vi "Kinect MAIN.vi"() -> ()   [LabVIEW 2014]
uses:
  Resources/Others/Control cluster.ctl
  <vilib>/University of Leeds/Kinesthesia Toolkit for Microsoft Kinect/_Polymorphic Configure/Event-Skeleton and Video.vi
  Kinect Global.vi
  <vilib>/University of Leeds/Kinesthesia Toolkit for Microsoft Kinect/_Polymorphic Read/Read-Skeleton and Video.vi
  <vilib>/University of Leeds/Kinesthesia Toolkit for Microsoft Kinect/_Polymorphic Close/Close-Skeleton and Video.vi
panel:
  out "Toggle Land/Take off":bool
  out "Hover":bool
  out "Control Cluster out":T1 {"Yaw Speed" scale=-1.0..1.0; "Vertical Speed" scale=-1.0..1.0; "Pitch" scale=-1.0..1.0; "Roll" scale=-1.0..1.0}
  out "pitch offset":dbl=0.15 format="%#_13g"
  out "Weak detect":bool=TRUE
  out "Colour data":picture
  out "error out":errorcluster
  out "Loop time":u32=25
  out "3D Picture":refnum<vi>(3d-picture)
  in  "stop":bool
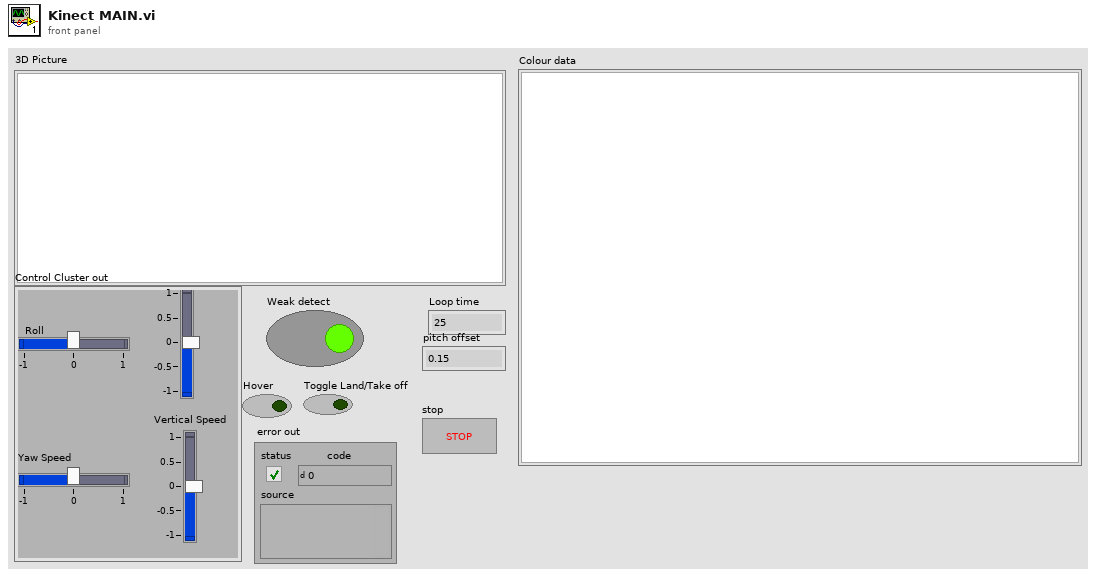
[diagram p1: front panel]
types:
  T1 = typedef "Control cluster.ctl" = cluster{"Roll":sgl, "Pitch":sgl, "Vertical Speed":sgl, "Yaw Speed":sgl}
  T2 = cluster{cluster{"reference out":refnum<k24>, "KinectSensors":refnum<k24>}, "get_Item":refnum<k24>}
  T3 = cluster{"Scene":refnum<vi>, "Joints":refnum<vi>[], "Bones":refnum<vi>[]}
  T4 = cluster{"reference out":refnum<k24>, "KinectSensors":refnum<k24>, "SkeletonStream":refnum<k24>, "ColorStream":refnum<k24>, refnum<k24>[], "get_Item":refnum<k24>}
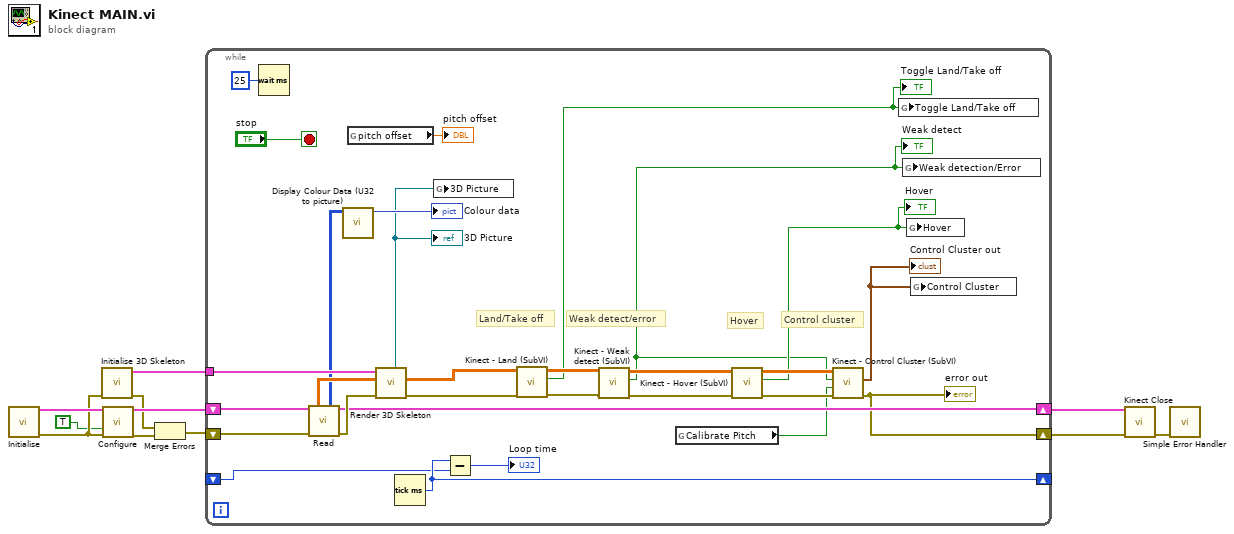
[diagram p0: block diagram]
diagram:
  n1 = call <vilib>:"Initialise.vi"() -> ("Kinect References out"=w11:T2, "error out"=w7:errorcluster)  [unwired: 14 in]
  n2 = call <vilib>:"Initialise 3D Skeleton.vi"("error in (no error)"=w7) -> ("error out"=w3:errorcluster, "Scene & Skeleton Refs"=w6:T3)  [unwired: 9 in]
  n3 = call-poly <vilib>:"Configure.vi"("Kinect References in"=w11, "Skeleton Smoothing"=TRUE, "error in"=w7) -> ("Kinect References out"=w10:T4, "error out"=w4:errorcluster)  [unwired: 11 in]
  n4 = Merge Errors(w3, w4) -> (w5:errorcluster)
  n5 = while {
    shift-right: [w24] -> w9
    shift-left: w10 -> [w29]
    shift-right: [w23] -> w8
    shift-left: w5 -> [w25]
    shift-right: [w40] -> _
    shift-left: _ -> [w39]
    tunnel: w6 -> [w28]
    stop <- "stop" stop-if-true
    # "Control cluster"
    # "Hover"
    # "Weak detect/error"
    # "Land/Take off"
    n6 = Wait (ms)(milliseconds to wait=u32 25) -> ()  [unwired: 1 out]
    n7 = call-poly <vilib>:"Read.vi"("Kinect References in"=w29, "error in (no error)"=w25) -> ("Primary Skeleton Array"=w22:dbl[][], "Colour output array (U24, RGB)"=w21:u32[][], "Kinect References out"=w24:T4, "error out"=w26:errorcluster)  [unwired: 9 in, 1 out]
    n8 = call <vilib>:"Display Colour Data (U32 to picture).vi"("Colour output array (U24, RGB)"=w21) -> ("new picture"=→"Colour data":picture)  [unwired: 10 in]
    n9 = global read "Kinect Global.vi" "pitch offset"() -> (→"pitch offset":dbl)
    n10 = call <vilib>:"Render 3D Skeleton.vi"("error in (no error)"=w26, "Array of Joint Positions"=w22, "Scene & Skeleton Refs In"=w28) -> ("error out"=w27:errorcluster, "Array of Joint Positions Out"=w34:dbl[][], "Scene Out"=w14:refnum<vi>)  [unwired: 5 in, 1 out]
    "3D Picture" <- w14
    n11 = Tick Count (ms)() -> (millisecond timer value=w40:u32)
    n12 = global write "Kinect Global.vi" "3D Picture"(w14) -> ()
    n13 = Subtract(x=w40, y=w39) -> (x-y=→"Loop time":u32)
    n14 = call "Kinect - Land (SubVI).vi"("error in (no error)"=w27, "Array of Joint Positions In"=w34) -> ("error out"=w36:errorcluster, "Toggle Land/Take off"=w18:bool, "Array of Joint Positions Out"=w35:dbl[][])  [unwired: 7 in]
    "Toggle Land/Take off" <- w18
    n15 = call "Kinect - Weak detect (SubVI).vi"("error in"=w36, "Array of Joint Positions In"=w35) -> ("error out"=w33:errorcluster, "Weak detect"=w16:bool, "Array of Joint Positions Out"=w32:dbl[][])  [unwired: 6 in]
    "Weak detect" <- w16
    n16 = global read "Kinect Global.vi" "Calibrate Pitch"() -> (w13:bool)
    n17 = call "Kinect - Hover (SubVI).vi"("error in"=w33, "Array of Joint Positions In"=w32) -> ("error out"=w31:errorcluster, "Boolean"=w17:bool, "Array of Joint Positions Out"=w20:dbl[][])  [unwired: 7 in]
    "Hover" <- w17
    n18 = call "Kinect - Control Cluster (SubVI).vi"("error in"=w31, "Calibrate Pitch"=w13, "Weak detect"=w16, "Array of Joint Positions in"=w20) -> ("error out"=w23:errorcluster, "Control Cluster out"=w30:T1)  [unwired: 4 in, 1 out]
    "error out" <- w23
    "Control Cluster out" <- w30
    n19 = global write "Kinect Global.vi" "Toggle Land/Take off"(w18) -> ()
    n20 = global write "Kinect Global.vi" "Weak detection/Error"(w16) -> ()
    n21 = global write "Kinect Global.vi" "Hover"(w17) -> ()
    n22 = global write "Kinect Global.vi" "Control Cluster"(w30) -> ()
  }
  n23 = call-poly <vilib>:"Kinect Close.vi"("Kinect References in"=w9, "error in"=w8) -> ("error out"=w2:errorcluster)  [unwired: 13 in]
  n24 = call <vilib>:"Simple Error Handler.vi"("error in (no error)"=w2) -> ()  [unwired: 4 in, 5 out]
